vi "Module Loop.vi"(8 "error in (no error)":errorcluster, 11 "DAQmxAO in":refnum<class "DAQmxAO.lvclass">) -> (0 "error out":errorcluster, 3 "DAQmxAO out":refnum<class "DAQmxAO.lvclass">)   [LabVIEW 2020, in "VolatusDAQ.lvlib" / "DAQmxAO.lvclass"]
uses:
  DAQmxAO.lvclass
  DAQmxAO.lvclass/DAQmxAO.ctl
  Volatus/Module/Module.lvclass
  messages/CmdAnalog/Class/Msg.lvclass
  lv-vecto/Vecto/Group/Group.lvclass
  lv-vecto/Vecto/Group DBL/Group DBL.lvclass
  VolatusData/Scaling/Scaling.lvclass
  <vilib>/DAQmx/write.llb/DAQmx Write (Analog 1D DBL NChan 1Samp).vi
  messages/CmdAnalogMultiple/Class/Msg.lvclass
  messages/CmdAnalog/Data.ctl
  messages/CmdAnalog/CmdAnalog.lvlib
  C:/dev/lv20CE/relink/lv-volatus/Volatus/Module/Module.lvclass
  C:/dev/lv20CE/relink/lv-volatus/VolatusDAQ/DAQmxAO/DAQmxAO.lvclass
  C:/dev/lv20CE/relink/lv-vecto/Vecto/Group/Group.lvclass
  C:/dev/lv20CE/relink/lv-vecto/Vecto/Group DBL/Group DBL.lvclass
  C:/dev/lv20CE/relink/lv-volatus/messages/CmdAnalog/Class/Msg.lvclass
  C:/dev/lv20CE/relink/lv-protoc/LV-Proto/Message/Message.lvclass
  C:/dev/lv20CE/relink/lv-volatus/messages/CmdAnalogMultiple/Class/Msg.lvclass
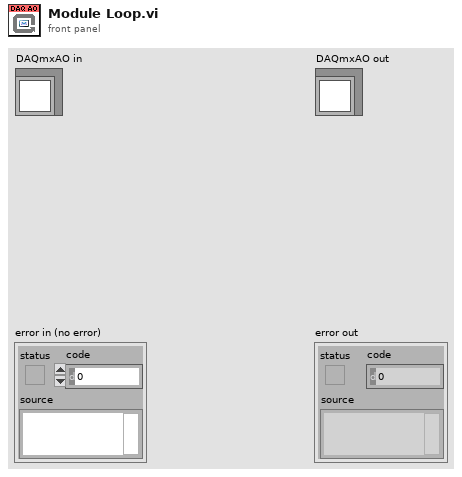
[diagram p1: front panel]
types:
  T1 = enum32{"Invalid", "Standard", "Closed", "Hidden", "Minimized", "Maximized"}
  T2 = typedef "CmdAnalog.lvlib/Data.ctl" = cluster{"channel":string, "value":dbl}
  T3 = typedef "CmdAnalogMultiple.lvlib/Data.ctl" = cluster{"values":T2[]}
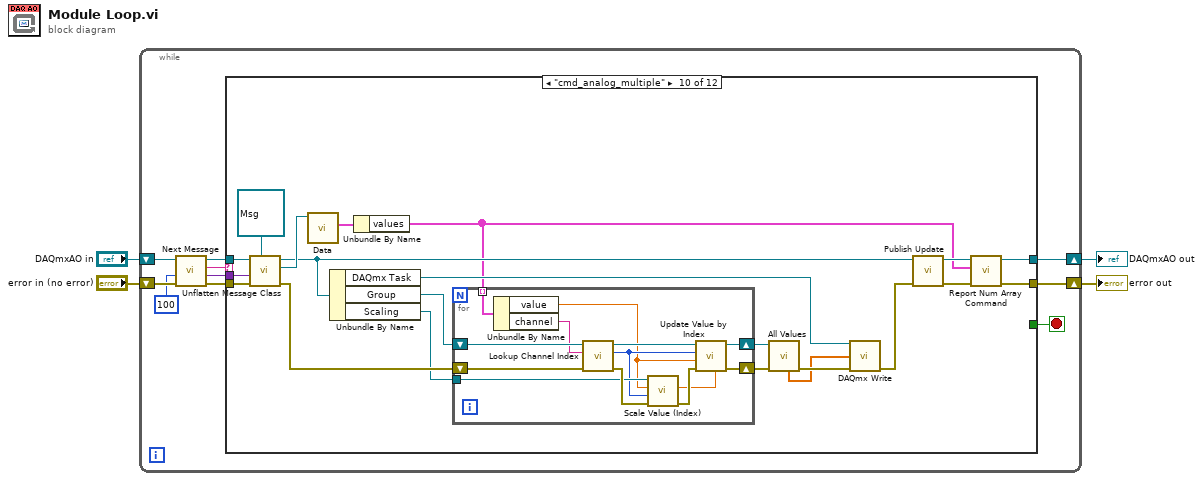
[diagram p0: block diagram]
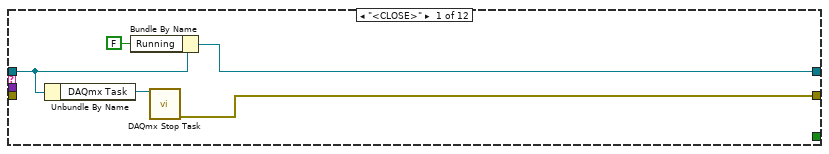
[diagram p2: hidden frame]
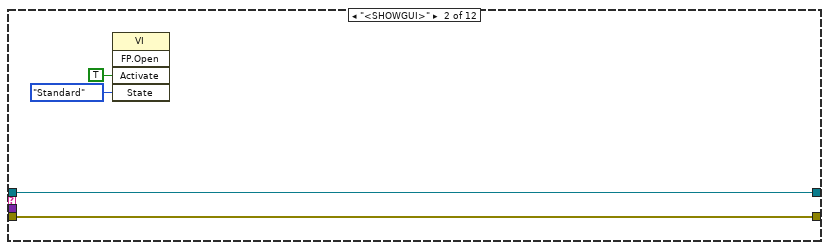
[diagram p3: hidden frame]
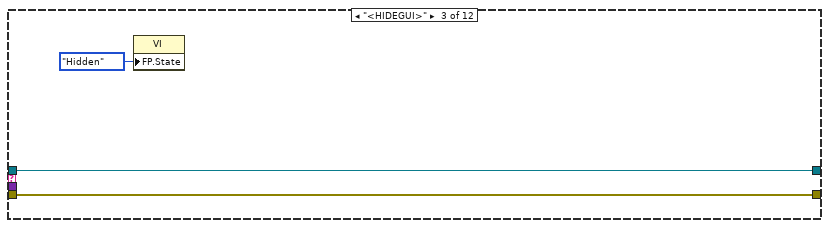
[diagram p4: hidden frame]
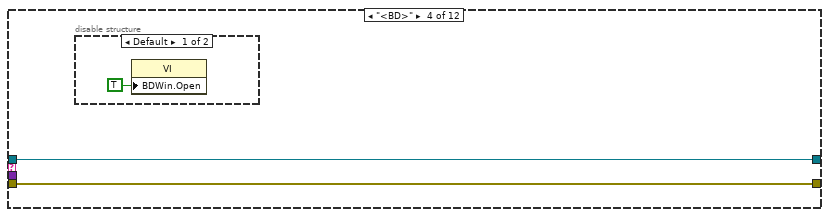
[diagram p5: hidden frame]
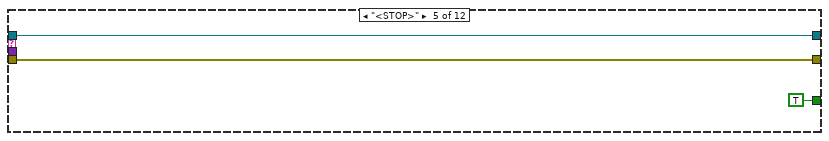
[diagram p7: hidden frame]
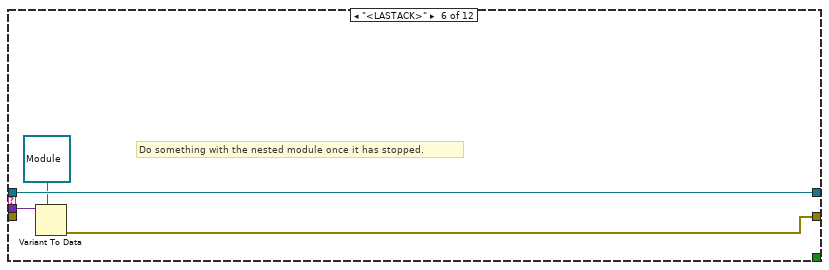
[diagram p8: hidden frame]
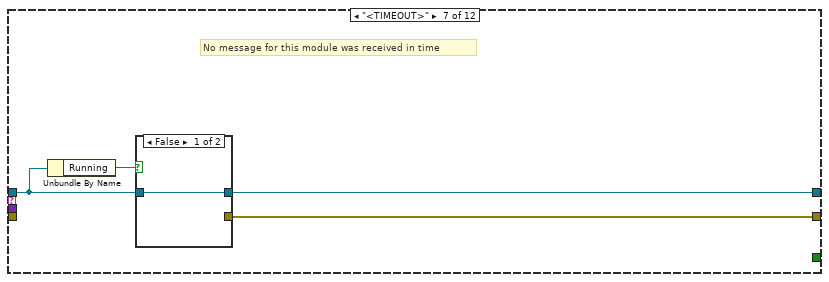
[diagram p9: hidden frame]
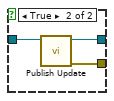
[diagram p10: hidden frame]
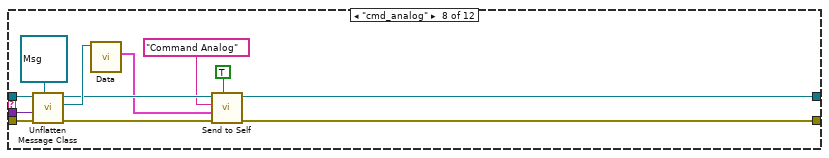
[diagram p11: hidden frame]
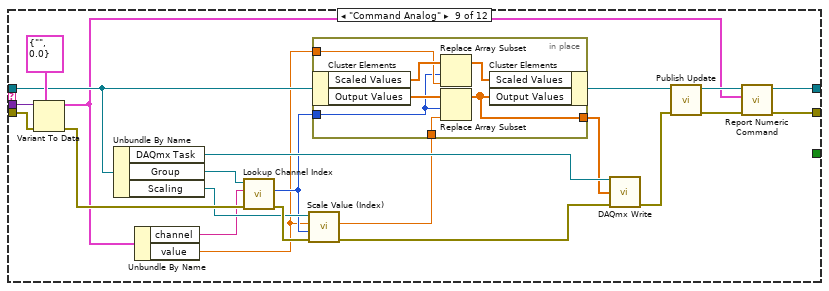
[diagram p12: hidden frame]
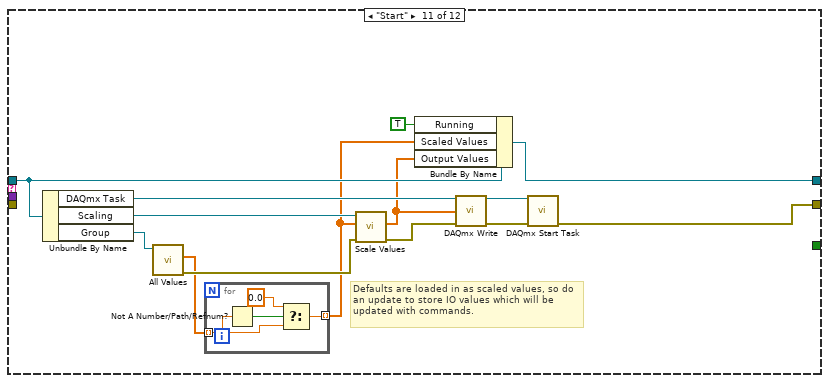
[diagram p13: hidden frame]
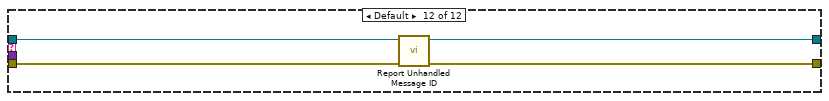
[diagram p14: hidden frame]
diagram:
  n1 = while {
    shift-right: [w9] -> w2
    shift-left: "DAQmxAO in" -> [w14]
    shift-right: [w8] -> w1
    shift-left: "error in (no error)" -> [w13]
    stop <- w7 stop-if-true
    n2 = call "Next Message.vi"("error in (no error)"=w13, "Timeout ms (-1)"=100, "Module in"=w14) -> ("error out"=w12:errorcluster, "Data"=w6:variant, "ID"=w11:string, "Module out"=w10:refnum<class "DAQmxAO.lvclass">)  [unwired: 5 in]
    n3 = case shown="\"cmd_analog_multiple\"" w11 {
      tunnel: w12 -> [_ w22 w25 w27 w31 _ _ w56 w70 w105 _ w141]
      tunnel: w10 -> [w19 w23 w26 w28 w32 w36 w40 w55 w68 w104 w132 w139]
      tunnel: [w17 w23 w26 w28 w32 w36 w39 w47 w58 w87 w124 w138] -> w9
      tunnel: [w15 w22 w25 w27 w31 w33 w38 w48 w60 w89 w121 w140] -> w8
      tunnel: [_ _ _ _ TRUE _ _ _ _ _ _ _] -> w7
      tunnel: w6 -> [_ _ _ _ _ w35 _ w54 w72 w103 _ _]
      frame "<CLOSE>" {
        n4 = Unbundle By Name(w19) -> ("DAQmx Task"=w18:refnum<k21>)
        n5 = Bundle By Name(cluster=w19, "Running"=FALSE) -> (w17:refnum<class "DAQmxAO.lvclass">)
        n6 = call <vilib>:"DAQmx Stop Task.vi"("task/channels in"=w18) -> ("error out"=w15:errorcluster)  [unwired: 13 in, 1 out]
      }
      frame "<SHOWGUI>" {
        n7 = invoke class="VI" method="FP.Open"("Activate"=TRUE ("Activate?"), "State"=T1."Standard") -> ()  [unwired: 3 in, 5 out]
      }
      frame "<HIDEGUI>" {
        n8 = property class="VI"("FP.State"=T1."Hidden" ("Front Panel Window:State")) -> ()  [unwired: 2 in, 2 out]
      }
      frame "<BD>" {
        n9 = disable-structure shown="Default" {
          frame condition #0 (active) {
            n10 = property class="VI"("BDWin.Open"=TRUE ("Block Diagram Window:Open")) -> ()  [unwired: 2 in, 2 out]
          }
          frame condition #1 {
          }
        }
      }
      frame "<STOP>" {
      }
      frame "<LASTACK>" {
        # "Do something with the nested module once it has stopped."
        n11 = Variant To Data(type=refnum<class "Module.lvclass"> refnum ("Volatus:Module"), Variant=w35) -> (error out=w33:errorcluster)  [unwired: 1 in, 1 out]
      }
      frame "<TIMEOUT>" {
        # "No message for this module was received in time"
        n12 = Unbundle By Name(w40) -> ("Running"=w37:bool)
        n13 = case shown="False" w37 {
          tunnel: w40 -> [w41 w44]
          tunnel: [w41 w43] -> w39
          tunnel: [_ w42] -> w38
          frame False {
          }
          frame True {
            n14 = call "Publish Update.vi"("DAQmxAO in"=w44) -> ("error out"=w42:errorcluster, "DAQmxAO out"=w43:refnum<class "DAQmxAO.lvclass">)  [unwired: 9 in]
          }
        }
      }
      frame "cmd_analog" {
        n15 = call "Unflatten Message Class.vi"("Message Type"=refnum<class "Msg.lvclass"> refnum ("CmdAnalog.lvlib:Msg.lvclass"), "error in (no error)"=w56, "Data"=w54, "Module in"=w55) -> ("error out"=w50:errorcluster, "Message"=w52:refnum<class "Msg.lvclass">, "Module out"=w51:refnum<class "DAQmxAO.lvclass">)  [unwired: 4 in, 1 out]
        n16 = call "Data.vi"("PB Msg Template in"=w52) -> ("Data"=w49:T2)  [unwired: 8 in, 2 out]
        n17 = call "Send to Self.vi"("High Priority (F)"=TRUE, "error in (no error)"=w50, "Data"=w49, "Message ID"="Command Analog", "Module in"=w51) -> ("error out"=w48:errorcluster, "Module out"=w47:refnum<class "DAQmxAO.lvclass">)  [unwired: 5 in]
      }
      frame "Command Analog" {
        n18 = Variant To Data(error in=w70, type=T2 {"channel"="", "value"=0.0} ("CmdAnalog"), Variant=w72) -> (data=w57:T2, error out=w78:errorcluster)
        n19 = Unbundle By Name(w68) -> ("DAQmx Task"=w74:refnum<k21>, "Group"=w76:refnum<class "Group DBL.lvclass">, "Scaling"=w75:refnum<class "Scaling.lvclass">)
        n20 = Unbundle By Name(w57) -> ("channel"=w73:string, "value"=w66:dbl)
        n21 = call "Lookup Channel Index.vi"("error in (no error)"=w78, "Channel Name"=w73, "Group in"=w76) -> ("error out"=w77:errorcluster, "Index"=w67:i32)  [unwired: 6 in, 1 out]
        n22 = call "Scale Value (Index).vi"("error in (no error)"=w77, "Index"=w67, "Value"=w66, "VolatusScaling in"=w75) -> ("error out"=w63:errorcluster, "Scaled Value"=w65:dbl)  [unwired: 5 in, 1 out]
        n23 = in-place {
          in-place-border: w67 -> [w82]
          in-place-border: w66 -> [w84]
          in-place-border: w65 -> [w81]
          in-place-border: [w79] -> w64
          n24 = in-place-cluster #1(w68) -> ("Scaled Values"=w85:dbl[], "Output Values"=w83:dbl[])
          n25 = Replace Array Subset(array=w85, new element=w84, index=w82) -> (w80:dbl[])
          n26 = Replace Array Subset(array=w83, new element=w81, index=w82) -> (w79:dbl[])
          n27 = in-place-cluster #1("Scaled Values"=w80, "Output Values"=w79) -> (w61:refnum<class "DAQmxAO.lvclass">)
        }
        n28 = call-poly <vilib>:"DAQmx Write.vi"("task/channels in"=w74, "data"=w64, "error in"=w63) -> ("error out"=w69:errorcluster)  [unwired: 10 in, 2 out]
        n29 = call "Publish Update.vi"("error in (no error)"=w69, "DAQmxAO in"=w61) -> ("error out"=w62:errorcluster, "DAQmxAO out"=w59:refnum<class "DAQmxAO.lvclass">)  [unwired: 8 in]
        n30 = call "Report Numeric Command.vi"("error in (no error)"=w62, "Command"=w57, "Module in"=w59) -> ("error out"=w60:errorcluster, "Module out"=w58:refnum<class "DAQmxAO.lvclass">)  [unwired: 7 in]
      }
      frame "cmd_analog_multiple" {
        n31 = call "Unflatten Message Class.vi"("Message Type"=refnum<class "Msg.lvclass"> refnum ("CmdAnalogMultiple.lvlib:Msg.lvclass"), "error in (no error)"=w105, "Data"=w103, "Module in"=w104) -> ("error out"=w106:errorcluster, "Message"=w94:refnum<class "Msg.lvclass">, "Module out"=w92:refnum<class "DAQmxAO.lvclass">)  [unwired: 4 in, 1 out]
        n32 = call "Data.vi"("PB Msg Template in"=w94) -> ("Data"=w93:T3)  [unwired: 8 in, 2 out]
        n33 = Unbundle By Name(w92) -> ("DAQmx Task"=w95:refnum<k21>, "Group"=w101:refnum<class "Group DBL.lvclass">, "Scaling"=w100:refnum<class "Scaling.lvclass">)
        n34 = Unbundle By Name(w93) -> ("values"=w86:T2[])
        n35 = for {
          tunnel: w100 -> [w115]
          shift-right: [w111] -> w99
          shift-left: w106 -> [w118]
          shift-right: [w110] -> w98
          shift-left: w101 -> [w117]
          tunnel: w86 -> [w109] mode=indexing
          n36 = Unbundle By Name(w109) -> ("value"=w107:dbl, "channel"=w108:string)
          n37 = call "Lookup Channel Index.vi"("error in (no error)"=w118, "Channel Name"=w108, "Group in"=w117) -> ("error out"=w119:errorcluster, "Index"=w114:i32, "Group out"=w116:refnum<class "Group DBL.lvclass">)  [unwired: 6 in]
          n38 = call "Scale Value (Index).vi"("error in (no error)"=w119, "Index"=w114, "Value"=w107, "VolatusScaling in"=w115) -> ("error out"=w113:errorcluster, "Scaled Value"=w112:dbl)  [unwired: 5 in, 1 out]
          n39 = call "Update Value by Index.vi"("Raw"=w112, "error in (no error)"=w113, "Scaled"=w107, "Index"=w114, "Group in"=w116) -> ("error out"=w111:errorcluster, "Group out"=w110:refnum<class "Group DBL.lvclass">)  [unwired: 5 in]
        }
        n40 = call "All Values.vi"("error in (no error)"=w99, "Group in"=w98) -> ("error out"=w97:errorcluster, "Raw"=w96:dbl[])  [unwired: 5 in, 3 out]
        n41 = call-poly <vilib>:"DAQmx Write.vi"("task/channels in"=w95, "data"=w96, "error in"=w97) -> ("error out"=w91:errorcluster)  [unwired: 10 in, 2 out]
        n42 = call "Publish Update.vi"("error in (no error)"=w91, "DAQmxAO in"=w92) -> ("error out"=w90:errorcluster, "DAQmxAO out"=w88:refnum<class "DAQmxAO.lvclass">)  [unwired: 8 in]
        n43 = call "Report Num Array Command.vi"("error in (no error)"=w90, "Command"=w86, "Module in"=w88) -> ("error out"=w89:errorcluster, "Module out"=w87:refnum<class "DAQmxAO.lvclass">)  [unwired: 7 in]
      }
      frame "Start" {
        # "Defaults are loaded in as scaled values, so do an update to store IO values which will be updated with commands."
        n44 = Unbundle By Name(w132) -> ("DAQmx Task"=w129:refnum<k21>, "Scaling"=w130:refnum<class "Scaling.lvclass">, "Group"=w131:refnum<class "Group DBL.lvclass">)
        n45 = call "All Values.vi"("Group in"=w131) -> ("error out"=w133:errorcluster, "Scaled"=w126:dbl[])  [unwired: 6 in, 3 out]
        n46 = for {
          tunnel: w126 -> [w136] mode=indexing
          tunnel: [w134] -> w123 mode=indexing
          n47 = Not A Number/Path/Refnum?(number/path/refnum=w136) -> (NaN/Path/Refnum?=w137:bool)
          n48 = Select(t=0.0, s=w137, f=w136) -> (s? t:f=w134:dbl)
        }
        n49 = call "Scale Values.vi"("error in (no error)"=w133, "Values"=w123, "VolatusScaling in"=w130) -> ("error out"=w125:errorcluster, "Scaled Values"=w122:dbl[])  [unwired: 6 in, 1 out]
        n50 = Bundle By Name(cluster=w132, "Running"=TRUE, "Scaled Values"=w123, "Output Values"=w122) -> (w124:refnum<class "DAQmxAO.lvclass">)
        n51 = call-poly <vilib>:"DAQmx Write.vi"("task/channels in"=w129, "data"=w122, "error in"=w125) -> ("task out"=w128:refnum<k21>, "error out"=w127:errorcluster)  [unwired: 10 in, 1 out]
        n52 = call <vilib>:"DAQmx Start Task.vi"("task/channels in"=w128, "error in"=w127) -> ("error out"=w121:errorcluster)  [unwired: 12 in, 1 out]
      }
      frame Default {
        n53 = call "Report Unhandled Message ID.vi"("error in (no error)"=w141, "Module in"=w139) -> ("error out"=w140:errorcluster, "Module out"=w138:refnum<class "DAQmxAO.lvclass">)  [unwired: 8 in]
      }
    }
  }
  "error out" <- w1
  "DAQmxAO out" <- w2
